vi "Clear Table.vi"(8 "error in":errorcluster, 10 "Confirm? (F)":bool, 11 "Table in":refnum<vi>) -> (0 "error out":errorcluster, 3 "T button?":bool)   [LabVIEW 2025, in "Automotive Ethernet Bus Monitor UI.lvlib"]
doc: "Clears the trace. Asks for clarification first if \"Confirm?\" is set to TRUE."
uses:
  Automotive Ethernet Bus Monitor UI.lvlib
  <vilib>/Utility/miscctls.llb/LVRowAndColumnTypeDef.ctl
  <vilib>/Utility/miscctls.llb/LVRowAndColumnUnsignedTypeDef.ctl
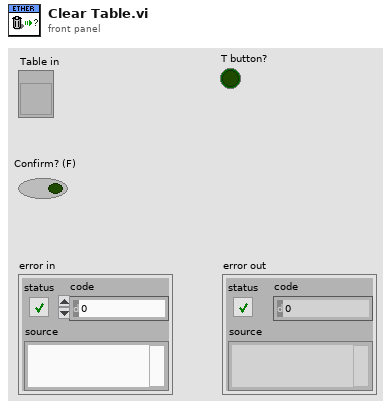
[diagram p1: front panel]
types:
  T1 = typedef "LVRowAndColumnUnsignedTypeDef.ctl" = cluster{"Row":u32, "Column":u32}
  T2 = typedef "LVRowAndColumnTypeDef.ctl" = cluster{"Row":i32, "Column":i32}
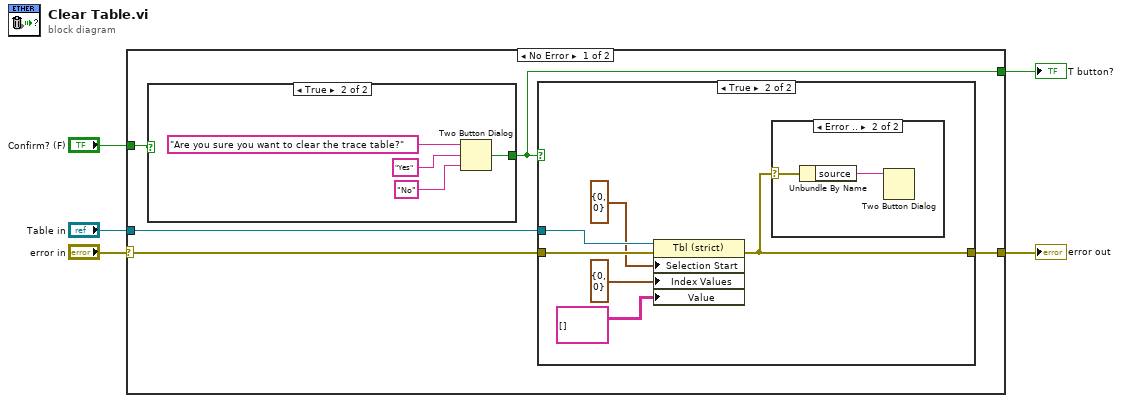
[diagram p0: block diagram]
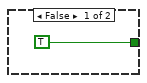
[diagram p2: hidden frame]
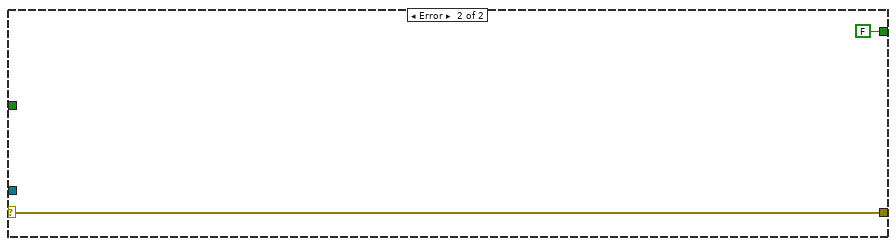
[diagram p5: hidden frame]
diagram:
  n1 = case shown="No Error" "error in" {
    selector: "error in" -> [w9 w26]
    tunnel: [w10 w26] -> w4
    tunnel: "Table in" -> [w8 _]
    tunnel: "Confirm? (F)" -> [w7 _]
    tunnel: [w6 FALSE ("T button?")] -> w1
    frame No Error {
      n2 = case shown="True" w7 {
        tunnel: [TRUE ("T button?") w15] -> w6
        frame False {
        }
        frame True {
          n3 = Two Button Dialog(message="Are you sure you want to clear the trace table?", 1:"No" ("F button name (\"Cancel\")"), 2:"Yes" ("T button name (\"OK\")")) -> (T button?=w15:bool)
        }
      }
      n4 = case shown="True" w6 {
        tunnel: w8 -> [_ w22]
        tunnel: [w16 w20] -> w10
        tunnel: w9 -> [w16 w21]
        frame False {
        }
        frame True {
          n5 = property class="Tbl (strict)"(reference=w22, error in=w21, "Selection Start"=T2 {"Row"=0, "Column"=0}, "Index Values"=T1 {"Row"=0, "Column"=0}, "Value"=string[][] [] ("Captured Data")) -> (error out=w20:errorcluster)  [unwired: 1 out]
          n6 = case shown="Error .." w20 {
            selector: w20 -> [_ w24]
            frame No Error {
            }
            frame Error {
              n7 = Unbundle By Name(w24) -> ("source"=w23:string)
              n8 = Two Button Dialog(message=w23) -> ()  [unwired: 2 in, 1 out]
            }
          }
        }
      }
    }
    frame Error {
    }
  }
  "error out" <- w4
  "T button?" <- w1
